vi "Create RPC Client Method.vi"(8 "error in (no error)":errorcluster, 10 "rpc method parameters":T1, 11 "library in":refnum<vi>) -> (0 "error out":errorcluster, 3 "library out":refnum<vi>)   [LabVIEW 2019, in "gRPC Template Creation Utility.lvlib"]
uses:
  gRPC Template Creation Utility.lvlib
  TypeDefs/RPC Method Parameters.ctl
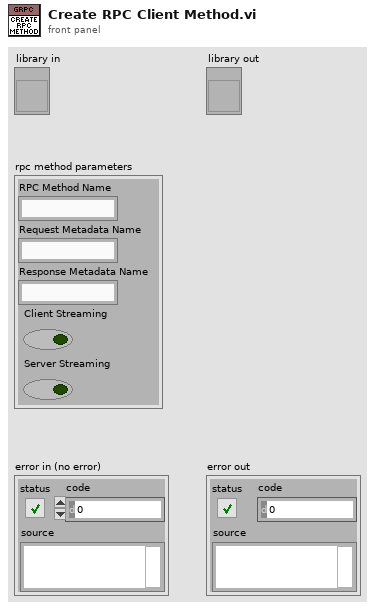
[diagram p1: front panel]
types:
  T1 = typedef "gRPC Template Creation Utility.lvlib/RPC Method Parameters.ctl" = cluster{"RPC Method Name":string, "Request Metadata Name":string, "Response Metadata Name":string, "Client Streaming":bool, "Server Streaming":bool}
  T2 = typedef "gRPC Template Creation Utility.lvlib/RPC Method Types.ctl" = enum16{"Unary", "Server Stream", "Client Stream", "Bidirectional Stream"}
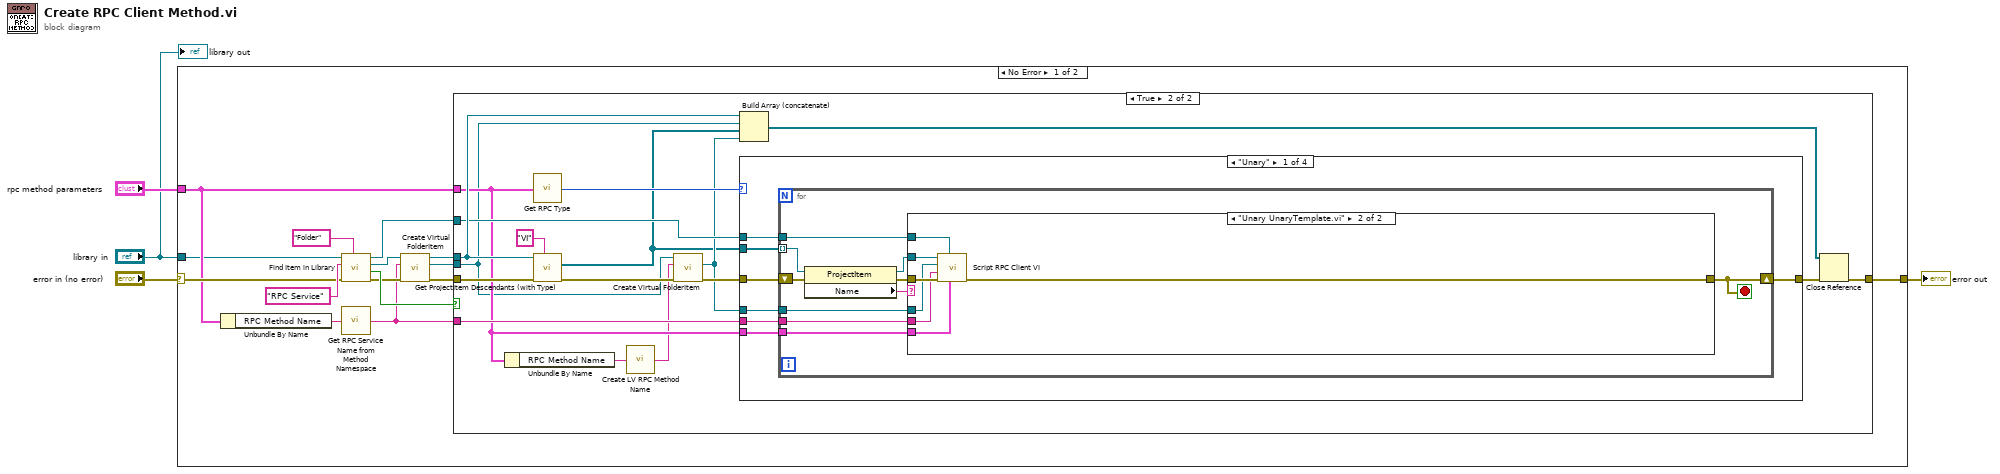
[diagram p0: block diagram]
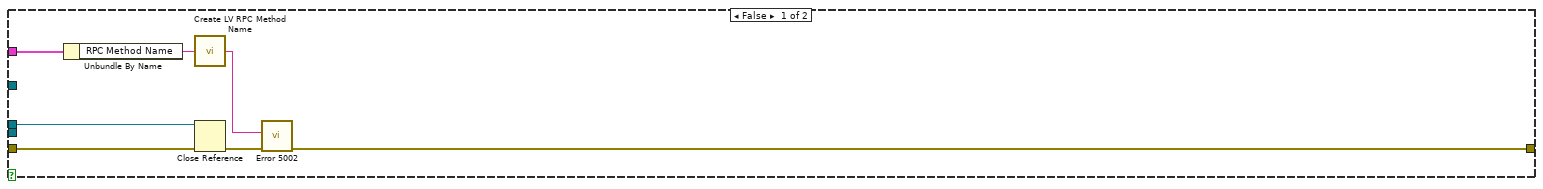
[diagram p2: hidden frame]
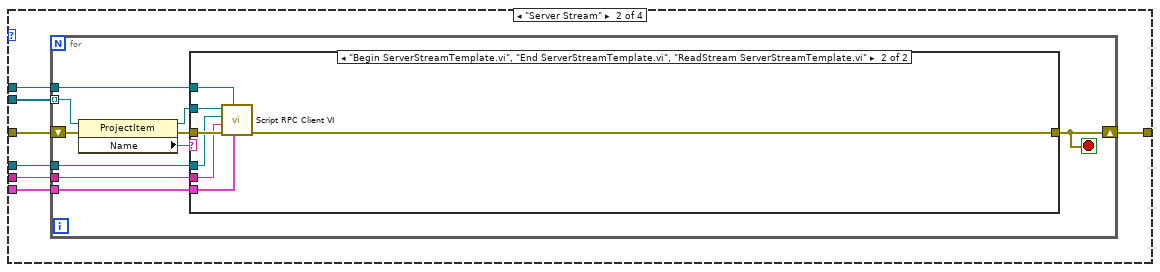
[diagram p4: hidden frame]
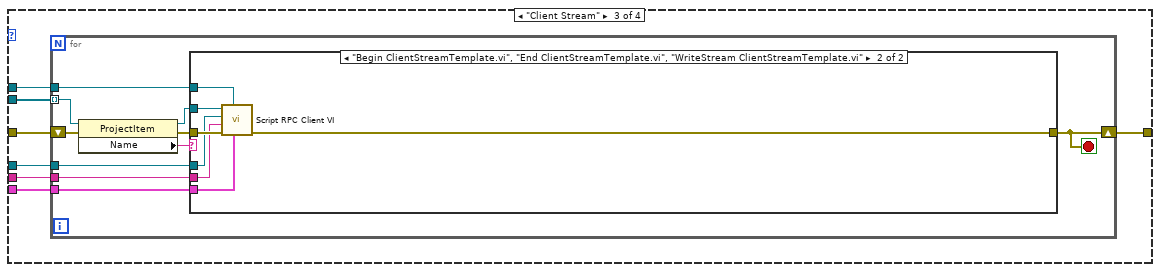
[diagram p6: hidden frame]
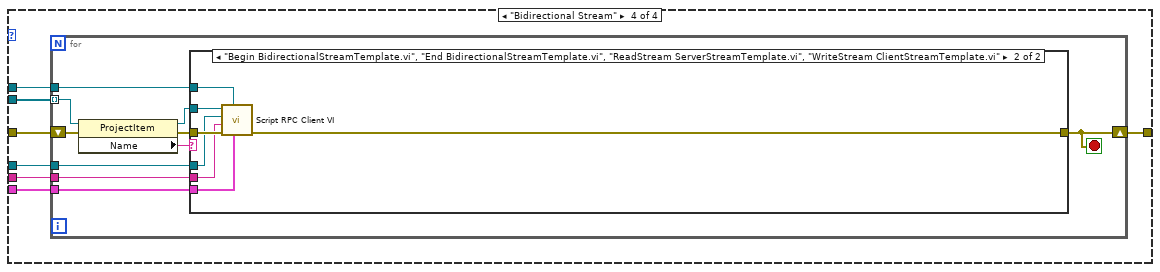
[diagram p8: hidden frame]
diagram:
  n1 = case shown="No Error" "error in (no error)" {
    selector: "error in (no error)" -> [w16 w144]
    tunnel: "library in" -> [w7 _]
    tunnel: [w17 w144] -> w4
    tunnel: "rpc method parameters" -> [w8 _]
    frame No Error {
      n2 = Unbundle By Name(w8) -> ("RPC Method Name"=w14:string)
      n3 = call "Find Item in Library.vi"("Item Type"="Folder", "error in (no error)"=w16, "Item Name"="RPC Service", "Library item in"=w7) -> ("error out"=w13:errorcluster, "Found?"=w15:bool, "Project Item (Library Item)"=w11:refnum<vi>, "Library item out"=w6:refnum<vi>)  [unwired: 4 in]
      n4 = call "Get RPC Service Name from Method Namespace.vi"("RPC Method Name"=w14) -> ("RPC Service Name"=w9:string)
      n5 = call "Create Virtual FolderItem.vi"("error in (no error)"=w13, "Folder Name"=w9, "ProjectItem in"=w11) -> ("error out"=w12:errorcluster, "FolderItem reference out"=w10:refnum<vi>, "ProjectItem out"=w5:refnum<vi>)  [unwired: 5 in, 1 out]
      n6 = case shown="True" w15 {
        tunnel: w5 -> [w23 w38]
        tunnel: w12 -> [w21 w39]
        tunnel: [w22 w43] -> w17
        tunnel: w10 -> [_ w28]
        tunnel: w9 -> [_ w37]
        tunnel: w8 -> [w26 w32]
        tunnel: w6 -> [_ w35]
        frame False {
          n7 = Unbundle By Name(w26) -> ("RPC Method Name"=w25:string)
          n8 = call "Create LV RPC Method Name.vi"("Proto Parser RPC Method Name in"=w25) -> ("LV RPC Method Name out"=w24:string)
          n9 = Close Reference(reference=w23, error in (no error)=w21) -> (error out=w20:errorcluster)
          n10 = call "Error 5002.vi"("error in (no error)"=w20, "Method Name"=w24) -> ("error out"=w22:errorcluster)  [unwired: 9 in]
        }
        frame True {
          n11 = Unbundle By Name(w32) -> ("RPC Method Name"=w30:string)
          n12 = call "Get RPC Type.vi"("RPC Method Parameters"=w32) -> ("RPC Type"=w36:T2)
          n13 = call "Get ProjectItem Descendants (with Type).vi"("Type"="VI", "error in (no error)"=w39, "ProjectItem in"=w38) -> ("error out"=w34:errorcluster, "All Descendents"=w27:refnum<vi>[])  [unwired: 6 in, 1 out]
          n14 = call "Create LV RPC Method Name.vi"("Proto Parser RPC Method Name in"=w30) -> ("LV RPC Method Name out"=w29:string)
          n15 = call "Create Virtual FolderItem.vi"("error in (no error)"=w34, "Folder Name"=w29, "ProjectItem in"=w28) -> ("error out"=w33:errorcluster, "FolderItem reference out"=w31:refnum<vi>)  [unwired: 5 in, 2 out]
          n16 = Build Array (concatenate)(w38, w28, w27, w31) -> (w42:refnum<vi>[])
          n17 = case shown="\"Unary\"" w36 {
            tunnel: w27 -> [w50 w75 w100 w125]
            tunnel: w33 -> [w49 w74 w99 w124]
            tunnel: [w48 w73 w98 w123] -> w40
            tunnel: w31 -> [w47 w72 w97 w122]
            tunnel: w37 -> [w46 w71 w96 w121]
            tunnel: w32 -> [w45 w70 w95 w120]
            tunnel: w35 -> [w44 w69 w94 w119]
            frame "Unary" {
              n18 = for {
                tunnel: w50 -> [w60] mode=indexing
                tunnel: w47 -> [w57]
                shift-right: [w55] -> w48
                shift-left: w49 -> [w59]
                tunnel: w46 -> [w54]
                tunnel: w45 -> [w53]
                tunnel: w44 -> [w52]
                stop <- w55 stop-if-true
                n19 = property class="ProjectItem"(reference=w60, error in=w59) -> (reference out=w51:refnum<vi>, error out=w56:errorcluster, "Name"=w58:string)
                n20 = case shown="\"Unary UnaryTemplate.vi\"" w58 {
                  tunnel: w57 -> [_ w65]
                  tunnel: w56 -> [w61 w67]
                  tunnel: [w61 w66] -> w55
                  tunnel: w54 -> [_ w63]
                  tunnel: w53 -> [_ w62]
                  tunnel: w52 -> [_ w64]
                  tunnel: w51 -> [_ w68]
                  frame "None", Default {
                  }
                  frame "Unary UnaryTemplate.vi" {
                    n21 = call "Script RPC Client VI.vi"("rpc method parameters"=w62, "owning library"=w64, "error in (no error)"=w67, "rpc service name"=w63, "owning folder"=w65, "template project item"=w68) -> ("error out"=w66:errorcluster)  [unwired: 5 in]
                  }
                }
              }
            }
            frame "Server Stream" {
              n22 = for {
                tunnel: w75 -> [w85] mode=indexing
                tunnel: w72 -> [w82]
                shift-right: [w80] -> w73
                shift-left: w74 -> [w84]
                tunnel: w71 -> [w79]
                tunnel: w70 -> [w78]
                tunnel: w69 -> [w77]
                stop <- w80 stop-if-true
                n23 = property class="ProjectItem"(reference=w85, error in=w84) -> (reference out=w76:refnum<vi>, error out=w81:errorcluster, "Name"=w83:string)
                n24 = case shown="\"Begin ServerStreamTemplate.vi\", \"End ServerStreamTemplate.vi\", \"ReadStream ServerStreamTemplate.vi\"" w83 {
                  tunnel: w82 -> [_ w89]
                  tunnel: w81 -> [w86 w93]
                  tunnel: [w86 w92] -> w80
                  tunnel: w79 -> [_ w87]
                  tunnel: w78 -> [_ w88]
                  tunnel: w77 -> [_ w90]
                  tunnel: w76 -> [_ w91]
                  frame "None", Default {
                  }
                  frame "Begin ServerStreamTemplate.vi", "End ServerStreamTemplate.vi", "ReadStream ServerStreamTemplate.vi" {
                    n25 = call "Script RPC Client VI.vi"("rpc method parameters"=w88, "owning library"=w90, "error in (no error)"=w93, "rpc service name"=w87, "owning folder"=w89, "template project item"=w91) -> ("error out"=w92:errorcluster)  [unwired: 5 in]
                  }
                }
              }
            }
            frame "Client Stream" {
              n26 = for {
                tunnel: w100 -> [w110] mode=indexing
                tunnel: w97 -> [w107]
                shift-right: [w105] -> w98
                shift-left: w99 -> [w109]
                tunnel: w96 -> [w104]
                tunnel: w95 -> [w103]
                tunnel: w94 -> [w102]
                stop <- w105 stop-if-true
                n27 = property class="ProjectItem"(reference=w110, error in=w109) -> (reference out=w101:refnum<vi>, error out=w106:errorcluster, "Name"=w108:string)
                n28 = case shown="\"Begin ClientStreamTemplate.vi\", \"End ClientStreamTemplate.vi\", \"WriteStream ClientStreamTemplate.vi\"" w108 {
                  tunnel: w107 -> [_ w114]
                  tunnel: w106 -> [w111 w118]
                  tunnel: [w111 w117] -> w105
                  tunnel: w104 -> [_ w113]
                  tunnel: w103 -> [_ w112]
                  tunnel: w102 -> [_ w116]
                  tunnel: w101 -> [_ w115]
                  frame "None", Default {
                  }
                  frame "Begin ClientStreamTemplate.vi", "End ClientStreamTemplate.vi", "WriteStream ClientStreamTemplate.vi" {
                    n29 = call "Script RPC Client VI.vi"("rpc method parameters"=w112, "owning library"=w116, "error in (no error)"=w118, "rpc service name"=w113, "owning folder"=w114, "template project item"=w115) -> ("error out"=w117:errorcluster)  [unwired: 5 in]
                  }
                }
              }
            }
            frame "Bidirectional Stream" {
              n30 = for {
                tunnel: w125 -> [w135] mode=indexing
                tunnel: w122 -> [w132]
                shift-right: [w130] -> w123
                shift-left: w124 -> [w134]
                tunnel: w121 -> [w129]
                tunnel: w120 -> [w128]
                tunnel: w119 -> [w127]
                stop <- w130 stop-if-true
                n31 = property class="ProjectItem"(reference=w135, error in=w134) -> (reference out=w126:refnum<vi>, error out=w131:errorcluster, "Name"=w133:string)
                n32 = case shown="\"Begin BidirectionalStreamTemplate.vi\", \"End BidirectionalStreamTemplate.vi\", \"ReadStream ServerStreamTemplate.vi\", \"WriteStream ClientStreamTemplate.vi\"" w133 {
                  tunnel: w132 -> [_ w138]
                  tunnel: w131 -> [w136 w142]
                  tunnel: [w136 w141] -> w130
                  tunnel: w129 -> [_ w139]
                  tunnel: w128 -> [_ w140]
                  tunnel: w127 -> [_ w137]
                  tunnel: w126 -> [_ w143]
                  frame "None", Default {
                  }
                  frame "Begin BidirectionalStreamTemplate.vi", "End BidirectionalStreamTemplate.vi", "ReadStream ServerStreamTemplate.vi", "WriteStream ClientStreamTemplate.vi" {
                    n33 = call "Script RPC Client VI.vi"("rpc method parameters"=w140, "owning library"=w137, "error in (no error)"=w142, "rpc service name"=w139, "owning folder"=w138, "template project item"=w143) -> ("error out"=w141:errorcluster)  [unwired: 5 in]
                  }
                }
              }
            }
          }
          n34 = Close Reference(reference=w42, error in (no error)=w40) -> (error out=w43:errorcluster)
        }
      }
    }
    frame Error {
    }
  }
  "error out" <- w4
  "library out" <- "library in"
